vi "fifo_scratch.result.vi"(11 "in":u64) -> (3 "out":u64)   [LabVIEW 2020]
doc: "Scratch FPGA-target VI for the one-FIFO scripting experiment (2026-10-16). Starts as a U64 pass-through; the experiment helper drops a target-scoped FIFO Method Node onto this diagram by script."
uses:
  <vilib>/rvi/DataTransferAndStorage/Container/XNode/niFpgaContainer.xnode
  <vilib>/rvi/FIFO/Fifo_Resource/nirvififoEmulationWrite.vi
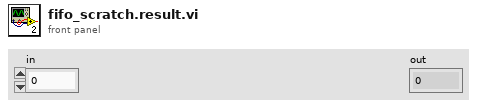
[diagram p1: front panel]
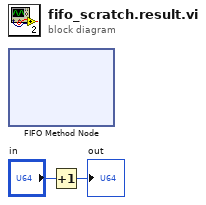
[diagram p0: block diagram]
diagram:
  n1 = xnode ("FIFO Method Node")() -> ()  [unwired: 3 in, 2 out]
  n2 = Increment(x="in") -> (x+1=→"out":u64)
